vi "test5-ChainNodeBroadcast.vi"(8 "error in (no error)":errorcluster, 11 "TestCase in":refnum<class "testcase-CSMChainMode.lvclass">) -> (0 "error out":errorcluster, 3 "TestCase out":refnum<class "testcase-CSMChainMode.lvclass">)   [LabVIEW 2017, in "testcase-CSMChainMode.lvclass"]
uses:
  testcase-CSMChainMode.lvclass
  b9a68168-9423-447a-be7f-8ac0ebad77aa.vi
  a50093c0-808a-49cf-b933-7f76f8d4e341.vi
  src/user.lib/_NEVSTOP/Communicable State Machine(CSM)/AdvanceAPI/CSM - Get Module Attribute.vi
  <vilib>/addons/_JKI Toolkits/VI Tester/TestCase.llb/TestCase.lvclass
  src/user.lib/_NEVSTOP/Communicable State Machine(CSM)/Communicable State Machine.lvlib
  C:/Program Files (x86)/National Instruments/LabVIEW 2017/vi.lib/addons/_JKI Toolkits/VI Tester/TestCase.llb/TestCase.lvclass
panel:
  out "LoopCount":i32
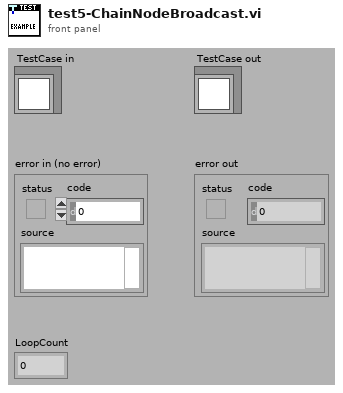
[diagram p1: front panel]
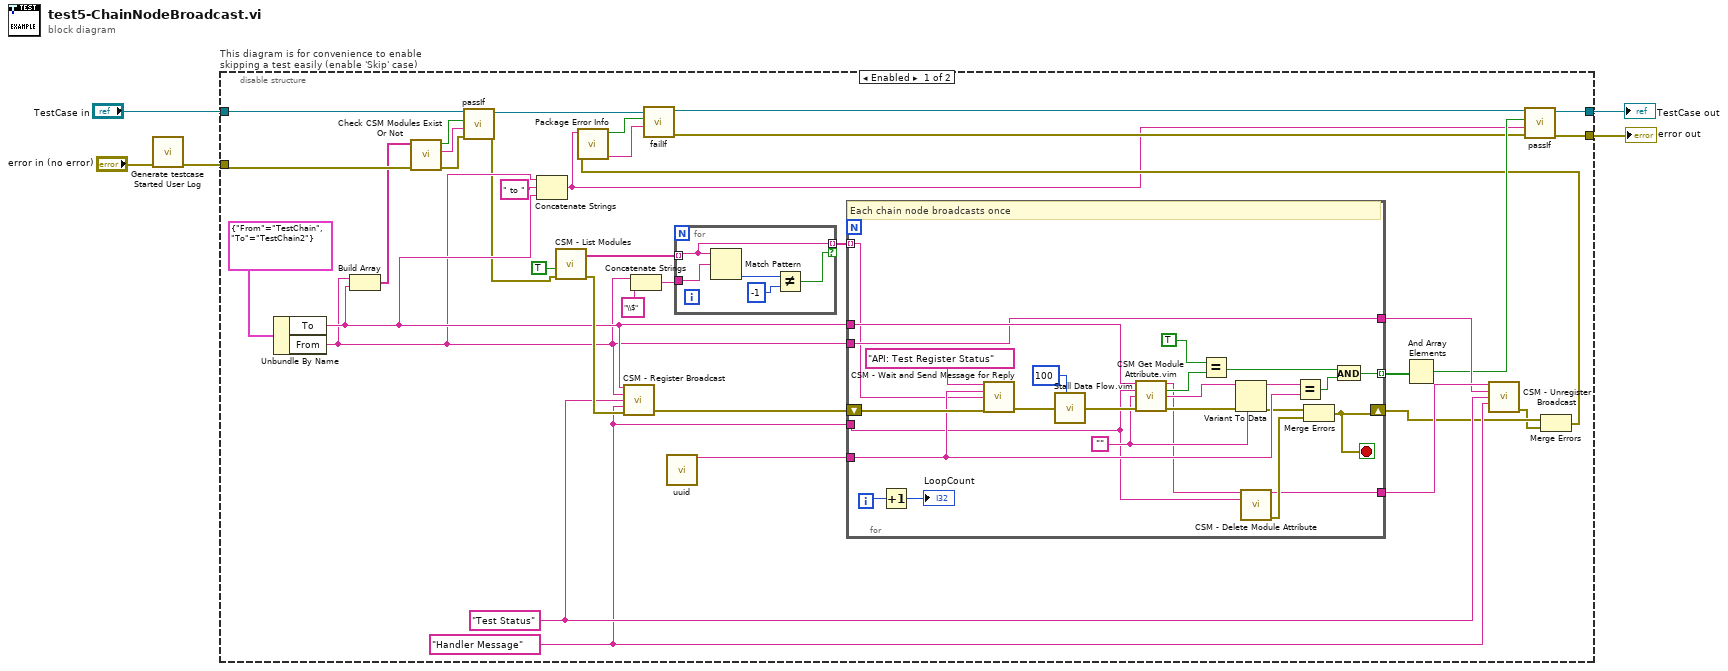
[diagram p0: block diagram]
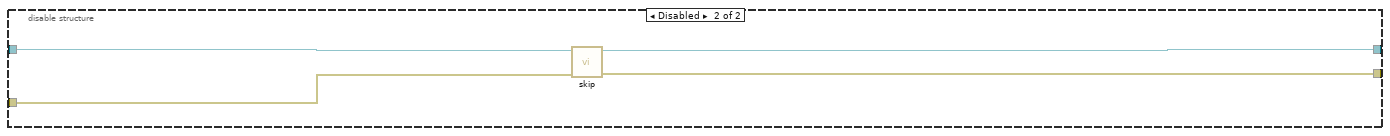
[diagram p2: hidden frame]
diagram:
  n1 = call "Generate testcase Started User Log.vi"("Error In"="error in (no error)") -> ("error out"=w1:errorcluster)  [unwired: 10 in]
  n2 = disable-structure "This diagram is for convenience to enable skipping a test easily (enable 'Skip' case)" shown="Enabled" {
    disable-tunnel: "TestCase in" -> [w15 w76]
    disable-tunnel: [w25 w74] -> w2
    disable-tunnel: [w24 w75] -> w4
    disable-tunnel: w1 -> [w13 w73]
    frame Enabled {
      w31 = "Handler Message" ("API (If \"\", Same as Trigger)")
      w32 = "Test Status" ("Trigger")
      n3 = Unbundle By Name(cluster{"From":string, "To":string} {"From"="TestChain", "To"="TestChain2"} ("Cluster")) -> ("To"=w11:string, "From"=w10:string)
      n4 = Build Array(w10, w11) -> (w12:string[])
      n5 = call "Check CSM Modules Exist Or Not.vi"("error in"=w13, "CSM names in"=w12) -> ("error out"=w20:errorcluster, "Debug string"=w21:string, "All Modules Exist?"=w22:bool)  [unwired: 7 in]
      n6 = call-dynamic "passIf.vi"("error in (no error)"=w20, "message (\"\")"=w21, "pass"=w22, "TestCase in"=w15) -> ("error out"=w9:errorcluster, "TestCase out"=w16:refnum<class "testcase-CSMChainMode.lvclass">)  [unwired: 6 in]
      n7 = Concatenate Strings(w10, " to " ("string"), w11) -> (w6:string)
      n8 = call "CSM - List Modules.vi"("Error In"=w9, "With Nodes? (F)"=TRUE) -> ("error out"=w34:errorcluster, "Module Names"=w37:string[])  [unwired: 8 in]
      n9 = call "CSM - Register Broadcast.vi"("CSM Name(Empty for Broadcast Event)"=w11, "Source CSM Name (* as Default)"=w10, "Trigger"=w32, "API (If \"\", Same as Trigger)"=w31, "Error In"=w34) -> ("error out"=w36:errorcluster)  [unwired: 9 in, 1 out]
      n10 = Concatenate Strings(w10, "\\$" ("string")) -> (w39:string)
      n11 = call "uuid.vi"() -> ("UUID"=w35:string)  [unwired: 11 in]
      n12 = for {
        tunnel: w37 -> [w70] mode=indexing
        tunnel: [w70] -> w33 mode=indexing if=w69
        tunnel: w39 -> [w68]
        n13 = Match Pattern(string=w70, regular expression=w68) -> (offset past match=w72:i32)  [unwired: 1 in, 3 out]
        n14 = Not Equal?(x=w72, y=-1) -> (x != y?=w69:bool)
      }
      n15 = for {
        tunnel: w35 -> [w53]
        tunnel: w33 -> [w43] mode=indexing
        tunnel: w11 -> [w60]
        tunnel: w31 -> [w49]
        shift-right: [w42] -> w28
        shift-left: w36 -> [w66]
        tunnel: w10 -> [w44]
        tunnel: [w46] -> w30
        tunnel: [w44] -> w29
        tunnel: [w45] -> w26 mode=indexing
        i -> [w65]
        stop <- w42 stop-if-true
        w55 = ""
        # "Each chain node broadcasts once"
        n16 = Increment(x=w65) -> (x+1=→"LoopCount":i32)
        n17 = call "CSM - Wait and Send Message for Reply.vi"("State"="API: Test Register Status", "Arguments (\"\")"=w53, "Target Module"=w43, "Error In (No Error)"=w66) -> ("error out"=w63:errorcluster)  [unwired: 8 in, 3 out]
        n18 = call "Stall Data Flow.vim"("value in"=w63, "milliseconds to wait"=u32 100) -> ("value out"=w61:errorcluster)  [unwired: 1 out]
        n19 = call "CSM Get Module Attribute.vim"("CSM Name"=w60, "Attribute"=w49, "Default Value (Empty Variant)"=w55, "Error In"=w61) -> ("CSM Name (Dup)"=w50:string, "Found"=w58:bool, "Value"=w56:string, "error out"=w57:errorcluster)  [unwired: 7 in, 1 out]
        n20 = Equal?(x=TRUE, y=w58) -> (x = y?=w51:bool)
        n21 = Variant To Data(error in=w57, type=w55, Variant=w56) -> (data=w54:string, error out=w48:errorcluster)
        n22 = call "CSM - Delete Module Attribute.vi"("CSM Name"=w50, "Attribute"=w49) -> ("CSM Name (Dup)"=w46:string, "error out"=w47:errorcluster)  [unwired: 10 in, 2 out]
        n23 = Equal?(x=w54, y=w53) -> (x = y?=w52:bool)
        n24 = Merge Errors(w48, w47) -> (w42:errorcluster)
        n25 = And(x=w51, y=w52) -> (x .and. y?=w45:bool)
      }
      n26 = And Array Elements(Boolean array=w26) -> (logical AND=w23:bool)
      n27 = call "CSM - Unregister Broadcast.vi"("CSM Name(Empty for Broadcast Event)"=w30, "Source CSM Name (* as Default)"=w29, "Trigger"=w32, "API (\"*\" as Default)"=w31) -> ("error out"=w27:errorcluster)  [unwired: 10 in, 1 out]
      n28 = Merge Errors(w28, w27) -> (w8:errorcluster)
      n29 = call "Package Error Info.vi"("error in"=w8, "String in"=w6) -> ("packed error info out"=w18:string, "error status"=w19:bool)  [unwired: 8 in]
      n30 = call-dynamic "failIf.vi"("message (\"\")"=w18, "fail"=w19, "TestCase in"=w16) -> ("error out"=w7:errorcluster, "TestCase out"=w14:refnum<class "testcase-CSMChainMode.lvclass">)  [unwired: 7 in]
      n31 = call-dynamic "passIf.vi"("error in (no error)"=w7, "message (\"\")"=w6, "pass"=w23, "TestCase in"=w14) -> ("error out"=w24:errorcluster, "TestCase out"=w25:refnum<class "testcase-CSMChainMode.lvclass">)  [unwired: 6 in]
    }
    frame Disabled {
      # "skip test result while test is under development"
      n32 = call <vilib>:"skip.vi"("error in (no error)"=w73, "TestCase in"=w76) -> ("error out"=w75:errorcluster, "TestCase out"=w74:refnum<class "testcase-CSMChainMode.lvclass">)  [unwired: 8 in]
    }
  }
  "error out" <- w4
  "TestCase out" <- w2
